vi "LaunchEventHandler.vi"(8 "error in (no error)":errorcluster, 11 "Navigator in":refnum<class "Navigator.lvclass">) -> (0 "error out":errorcluster, 3 "Navigator out":refnum<class "Navigator.lvclass">)   [LabVIEW 2024, in "Navigator.lvclass"]
doc: "Launch asynchronous event handling loop to handle Navigator events."
uses:
  Navigator.lvclass
  EventHandler.vi
  Navigator.lvclass/Navigator.ctl
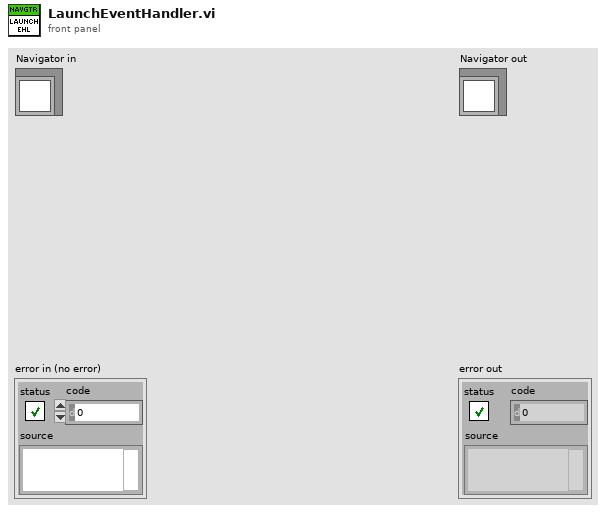
[diagram p1: front panel]
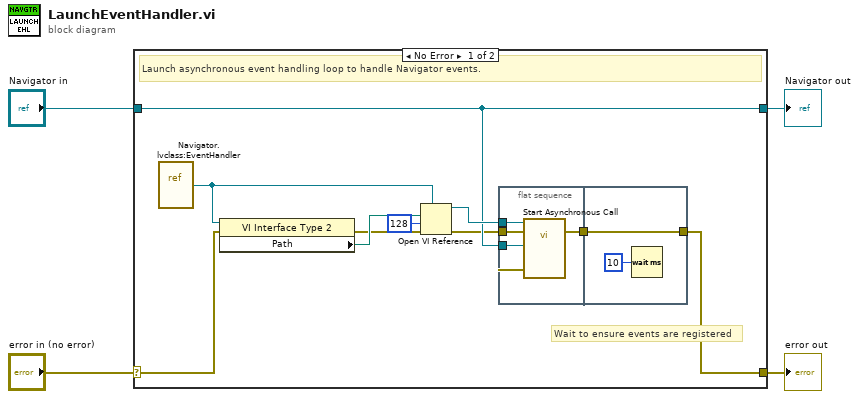
[diagram p0: block diagram]
diagram:
  n1 = case shown="No Error" "error in (no error)" {
    selector: "error in (no error)" -> [w10 w22]
    tunnel: [w9 w22] -> w3
    tunnel: [w8 w21] -> w1
    tunnel: "Navigator in" -> [w8 w21]
    frame No Error {
      # "Wait to ensure events are registered"
      # "Launch asynchronous event handling loop to handle Navigator events."
      n2 = vi-ref "Navigator.lvclass:EventHandler.vi"() -> (w14:refnum<vi>)
      n3 = property class="VI Interface Type 2"(reference=w14, error in=w10) -> (error out=w11:errorcluster, "Path"=w13:path)  [unwired: 1 out]
      n4 = Open VI Reference(type specifier VI Refnum (for type only)=w14, vi path=w13, options=128, error in (no error)=w11) -> (vi reference=w12:refnum<vi>, error out=w7:errorcluster)  [unwired: 2 in]
      n5 = flat-sequence {
        tunnel: w12 -> [w18]
        tunnel: w8 -> [w16]
        tunnel: w7 -> [w15]
        tunnel: [w17] -> w6
        tunnel: [w20] -> w9
        tunnel: w6 -> [w20]
        frame #0 {
          n6 = call-by-ref "Start Asynchronous Call"(reference=w18, error in=w15, 8:"error in (no error)"=w15, "Navigator in"=w16) -> (error out=w17:errorcluster)  [unwired: 8 in, 3 out]
        }
        frame #1 {
          n7 = Wait (ms)(milliseconds to wait=u32 10) -> ()  [unwired: 1 out]
        }
      }
    }
    frame Error {
    }
  }
  "error out" <- w3
  "Navigator out" <- w1
